vi "optical_grab2.vi"() -> ()   [LabVIEW 2025]
uses:
  <vilib>/vision/driver/NI_Vision_Acquisition_Software.lvlib
  <resource>/objmgr/imaqdx.rc
panel:
  out "file path out":path
  out "Time bw Frames":u32
  out "max value":u16
  out "Image Pixels (U16)":u16[][](array[numeric])
  out "Image Preview":T1(plugin-control)
  out "error out":errorcluster
  out "FPS":u32
  in  "Output Folder":path=path "../data/raw/test_6"
  in  "Stop":bool
  in  "Camera Name":refnum<k21> caption="IMAQdx Session"
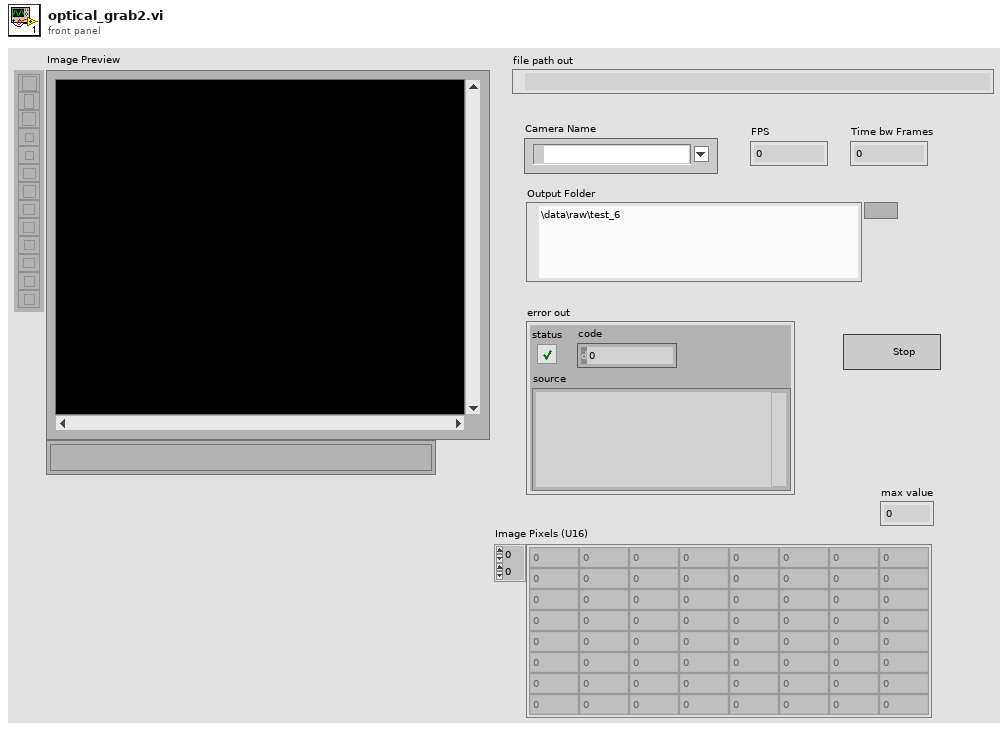
[diagram p1: front panel]
types:
  T1 = typedef "IMAQ Image.ctl" = refnum<image>
  T2 = typedef "Image Type" = u32
  T3 = typedef "IMAQdx.ctl" = refnum<k21>
  T4 = enum16{"open", "open or create", "create or replace", "create", "open (read-only)"}
  T5 = enum16{"big-endian, network order", "native, host order", "little-endian"}
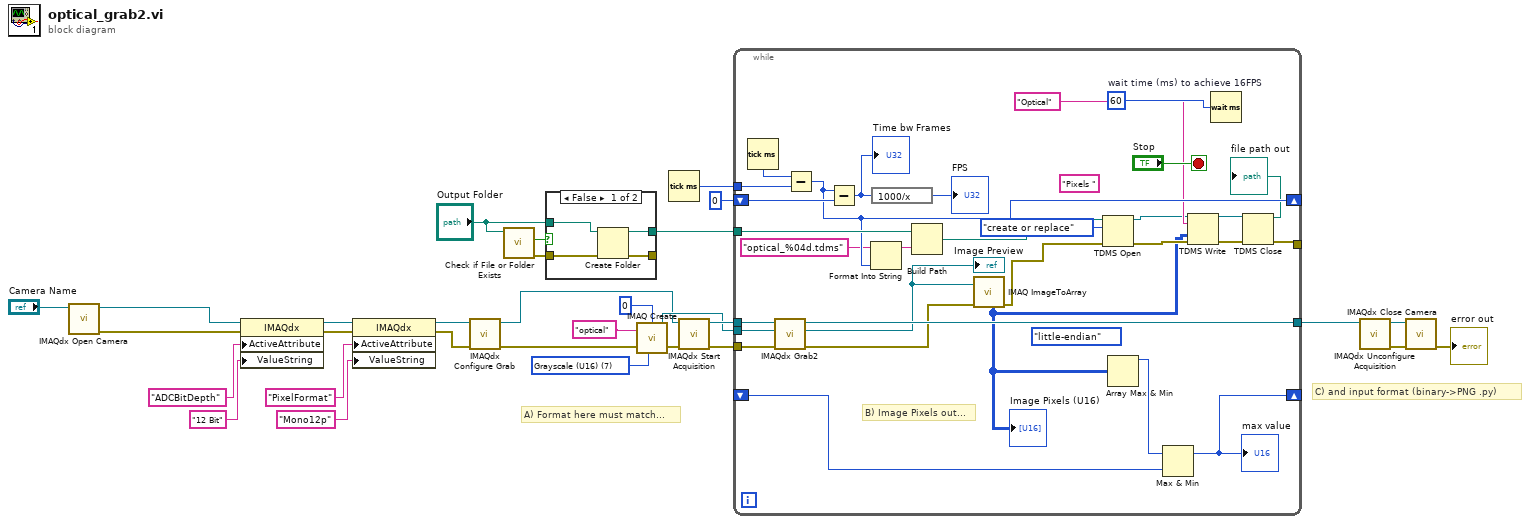
[diagram p0: block diagram]
diagram:
  w22 = T2 7 items=["Grayscale (U8)", "Grayscale (I16)", "Grayscale (SGL)", "Complex (CSG)", "RGB (U32)", "HSL (U32)", "RGB (U64)", "Grayscale (U16)"] ("Image Type")
  # "C) and input format (binary->PNG .py)"
  # "A) Format here must match..."
  n1 = call <vilib>:"IMAQdx Open Camera.vi"("Session In"="Camera Name") -> ("error out"=w18:errorcluster, "Session Out"=w19:T3)  [unwired: 9 in]
  n2 = property class="IMAQdx"(reference=w19, error in=w18, "ActiveAttribute"="ADCBitDepth", "ValueString"="12 Bit") -> (reference out=w6:T3, error out=w4:errorcluster)
  n3 = property class="IMAQdx"(reference=w6, error in=w4, "ActiveAttribute"="PixelFormat", "ValueString"="Mono12p" ("ActiveAttribute")) -> (reference out=w5:T3, error out=w3:errorcluster)
  n4 = call <vilib>:"IMAQdx Configure Grab.vi"("error in"=w3, "Session In"=w5) -> ("error out"=w10:errorcluster, "Session Out"=w9:T3)  [unwired: 8 in]
  n5 = call <vilib>:"Check if File or Folder Exists.vi"("path"="Output Folder") -> ("error out"=w28:errorcluster, "file or folder exists?"=w30:bool)  [unwired: 8 in, 1 out]
  n6 = case shown="False" w30 {
    tunnel: "Output Folder" -> [w34 w36]
    tunnel: [w33 w36] -> w27
    tunnel: w28 -> [w32 w35]
    tunnel: [w31 w35] -> _
    frame False {
      n7 = Create Folder(path (use dialog)=w34, error in=w32) -> (created path=w33:path, error out=w31:errorcluster)  [unwired: 1 in, 1 out]
    }
    frame True {
    }
  }
  n8 = call "IMAQ Create"("Border Size"=0, "Image Name"="optical", "Image Type"=w22, "error in (no error)"=w10) -> ("New Image"=w13:T1, "error out"=w12:errorcluster)  [unwired: 1 in]
  n9 = Tick Count (ms)() -> (millisecond timer value=w26:u32)
  n10 = call <vilib>:"IMAQdx Start Acquisition.vi"("error in"=w12, "Session In"=w9) -> ("error out"=w11:errorcluster, "Session Out"=w20:T3)  [unwired: 8 in]
  n11 = while {
    tunnel: w27 -> [w67]
    tunnel: w26 -> [w65]
    shift-right: [w63] -> _
    shift-left: u32 0 -> [w64]
    tunnel: w20 -> [w59]
    tunnel: w13 -> [w58]
    tunnel: w11 -> [w57]
    tunnel: [w55] -> w17
    shift-right: [w50] -> _
    shift-left: _ -> [w51]
    tunnel: [w46] -> _
    stop <- "Stop" stop-if-true
    (unwired) "Pixels "
    w49 = u32 60  # wait time (ms) to achieve 16FPS
    (unwired) T5."little-endian" ("byte order (0:big-endian, network order)")
    # "B) Image Pixels out..."
    n12 = Tick Count (ms)() -> (millisecond timer value=w66:u32)
    n13 = call <vilib>:"IMAQdx Grab2.vi"("error in"=w57, "Image In"=w58, "Session In"=w59) -> ("error out"=w53:errorcluster, "Image Out"=w54:T1, "Session Out"=w55:T3)  [unwired: 5 in, 1 out]
    "Image Preview" <- w54
    n14 = Subtract(x=w66, y=w65) -> (x-y=w63:u32)
    n15 = Subtract(x=w63, y=w64) -> (x-y=w48:u32)
    "Time bw Frames" <- w48
    n16 = Format Into String(format string="optical_%04d.tdms", w63) -> (resulting string=w62:string)  [unwired: 2 in, 1 out]
    n17 = expression code="1000/x"(w48) -> (→"FPS":u32)
    n18 = Build Path(base path=w67, name or relative path=w62) -> (appended path=w42:path)
    n19 = call "IMAQ ImageToArray"("error in (no error)"=w53, "Image"=w54) -> ("Image Pixels (U16)"=w37:u16[][], "error out"=w40:errorcluster)  [unwired: 2 in, 3 out]
    "Image Pixels (U16)" <- w37
    n20 = TDMS Open(8:w40, 10:T4."create or replace" ("operation (0:open)"), 11:w42) -> (0:w39:errorcluster, 3:w41:refnum<k34>)  [unwired: 4 in]
    n21 = Array Max & Min(array=w37) -> (max value=w52:u16)  [unwired: 3 out]
    n22 = Max & Min(x=w52, y=w51) -> (max(x,y)=w50:u16)  [unwired: 1 out]
    "max value" <- w50
    n23 = TDMS Write(0:w41, 5:"Optical", 9:w37, 11:w39) -> (4:w44:refnum<k34>, 15:w47:errorcluster)  [unwired: 2 in, 2 out]
    n24 = Wait (ms)(milliseconds to wait=w49) -> ()  [unwired: 1 out]
    n25 = TDMS Close(8:w47, 11:w44) -> (0:w46:errorcluster, 3:→"file path out":path)
  }
  n26 = call <vilib>:"IMAQdx Unconfigure Acquisition.vi"("Session In"=w17) -> ("error out"=w15:errorcluster, "Session Out"=w16:T3)  [unwired: 9 in]
  n27 = call <vilib>:"IMAQdx Close Camera.vi"("error in"=w15, "Session In"=w16) -> ("error out"=→"error out":errorcluster)  [unwired: 9 in]
